vi "Create Oneof Message Converter Skeletons.vi"(8 "error in (no error)":errorcluster, 10 "Message parameters":T1[](array[typedef]), 11 "Library in":refnum<vi>) -> (0 "error out":errorcluster, 3 "Library out":refnum<vi>)   [LabVIEW 2019, in "gRPC Template Creation Utility.lvlib"]
uses:
  gRPC Template Creation Utility.lvlib
  TypeDefs/Message Metadata (Scripting).ctl
  TypeDefs/Message Element Metadata (Scripting).ctl
  TypeDefs/Message Element Type.ctl
  OneOf Constants/OneOfConstantsEnum.ctl
  <vilib>/Utility/traverseref.llb/TRef TravTarget.ctl
  <vilib>/Utility/traverseref.llb/VI Scripting - Traverse.lvlib
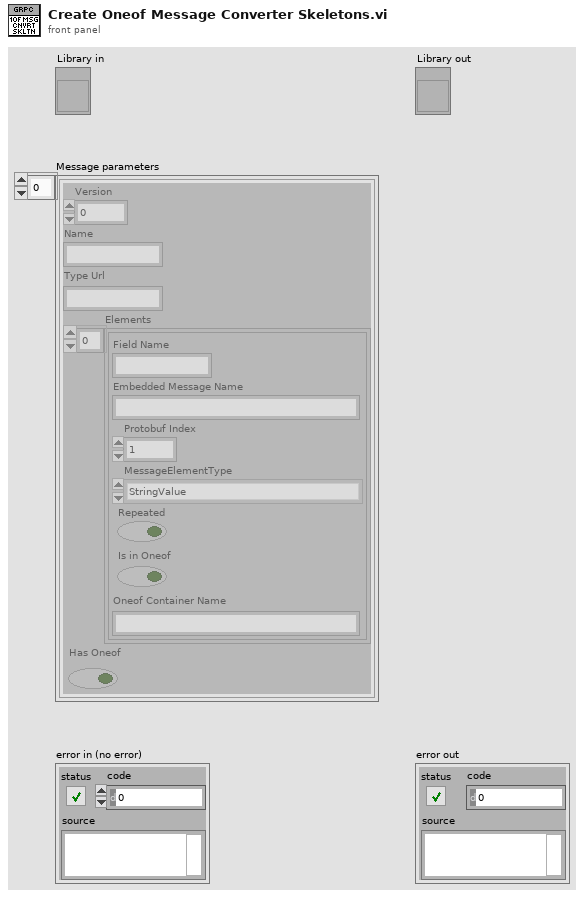
[diagram p1: front panel]
types:
  T1 = typedef "gRPC Template Creation Utility.lvlib/Message Metadata (Scripting).ctl" = cluster{"Version":i32, "Name":string, "Type Url":string, "Elements":T2[], "Has Oneof":bool}
  T2 = typedef "gRPC Template Creation Utility.lvlib/Message Element Metadata (Scripting).ctl" = cluster{"Field Name":string, "Embedded Message Name":string, "Protobuf Index":i32, "MessageElementType":T3, "Repeated":bool, "Is in Oneof":bool, "Oneof Container Name":string}
  T3 = typedef "gRPC Template Creation Utility.lvlib/Message Element Type.ctl" = enum32{"Int32Value", "FloatValue", "DoubleValue", "BoolValue", "StringValue", "MessageValue", "Int64Value", "UInt32Value", "UInt64Value", "EnumValue", "Bytes", "Fixed64", "Fixed32", "SFixed64", "SFixed32", "SInt64", "SInt32"}
  T4 = typedef "gRPC Template Creation Utility.lvlib/OneOfConstantsEnum.ctl" = enum16{"FlatToRichVIPrefix", "RichToFlatVIPrefix", "FlatTypeDefSuffix"}
  T5 = typedef "TRef TravTarget.ctl" = enum16{"FP", "BD", "Other"}
  T6 = enum32{"invalid scope", "public", "private", "protected", "community"}
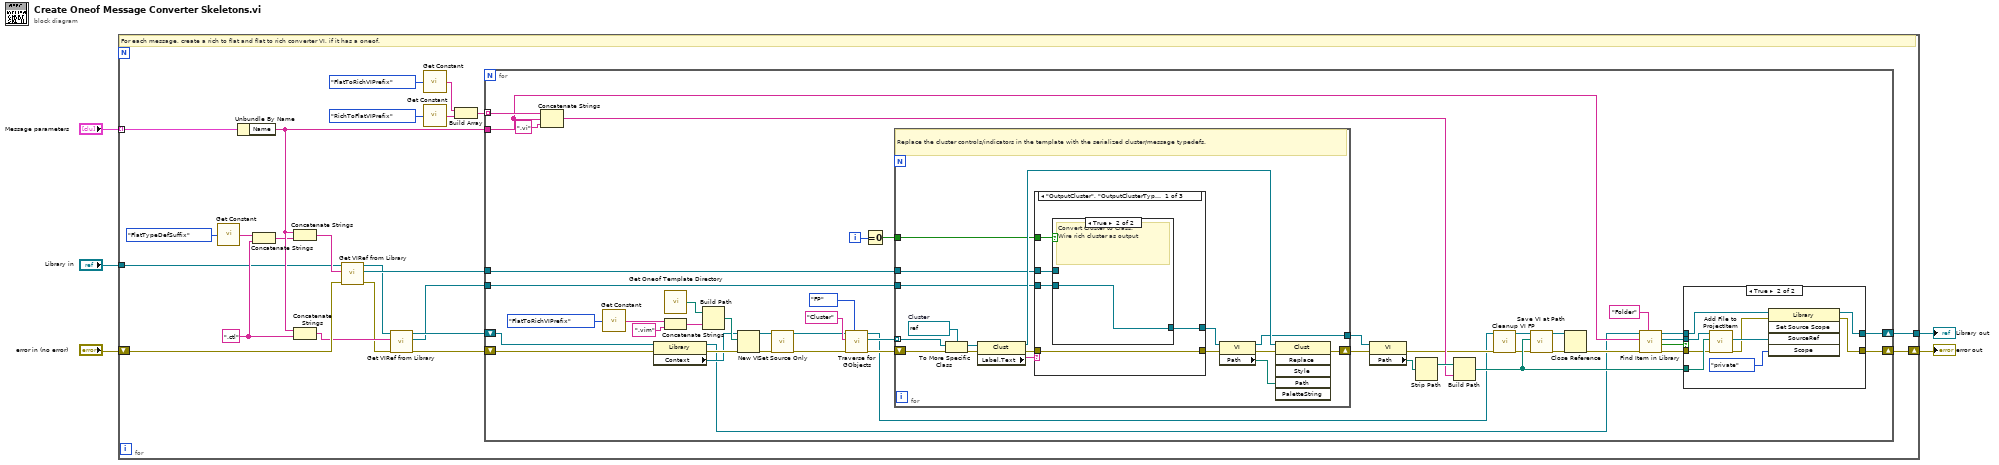
[diagram p0: block diagram]
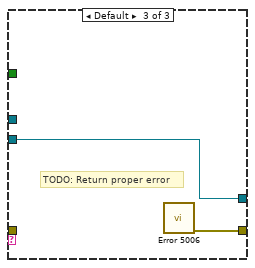
[diagram p6: hidden frame]
diagram:
  n1 = for {
    tunnel: "Message parameters" -> [w28] mode=indexing
    shift-right: [w23] -> w3
    shift-left: "error in (no error)" -> [w27]
    tunnel: "Library in" -> [w11]
    tunnel: [w25] -> w5
    w12 = ".ctl" ("string")
    # "For each message, create a rich to flat and flat to rich converter VI, if it has a oneof."
    n2 = call "Get Constant.vi"("Selection"=OneOfConstantsEnum."FlatTypeDefSuffix") -> ("String"=w18:string)
    n3 = Unbundle By Name(w28) -> ("Name"=w21:string)
    n4 = Concatenate Strings(w18, w12) -> (w20:string)
    n5 = Concatenate Strings(w21, w20) -> (w24:string)
    n6 = Concatenate Strings(w21, w12) -> (w22:string)
    n7 = call "Get VIRef from Library.vi"("error in (no error)"=w27, "Item Name"=w24, "Library"=w11) -> ("error out"=w7:errorcluster, "VIref out"=w9:refnum<vi>, "Library"=w8:refnum<vi>)  [unwired: 5 in, 1 out]
    n8 = call "Get VIRef from Library.vi"("error in (no error)"=w7, "Item Name"=w22, "Library"=w8) -> ("error out"=w6:errorcluster, "VIref out"=w10:refnum<vi>, "Library"=w26:refnum<vi>)  [unwired: 5 in, 1 out]
    n9 = call "Get Constant.vi"("Selection"=OneOfConstantsEnum."FlatToRichVIPrefix") -> ("String"=w15:string)
    n10 = call "Get Constant.vi"("Selection"=OneOfConstantsEnum."RichToFlatVIPrefix") -> ("String"=w14:string)
    n11 = Build Array(w15, w14) -> (w13:string[])
    n12 = for {
      tunnel: w9 -> [w74]
      tunnel: w21 -> [w51]
      tunnel: w10 -> [w68]
      shift-right: [w34] -> w25
      shift-left: w26 -> [w33]
      shift-right: [w55] -> w23
      shift-left: w6 -> [w32]
      tunnel: w13 -> [w62] mode=indexing
      i -> [w61]
      n13 = Concatenate Strings(w62, w51, ".vi" ("string")) -> (w69:string)
      n14 = call "Get Constant.vi"("Selection"=OneOfConstantsEnum."FlatToRichVIPrefix") -> ("String"=w49:string)
      n15 = property class="Library"(reference=w33, error in=w32) -> (reference out=w29:refnum<vi>, error out=w31:errorcluster, "Context"=w30:refnum<vi>)
      n16 = call "Get Oneof Template Directory.vi"() -> ("appended path"=w52:path)
      n17 = Concatenate Strings(w49, ".vim" ("string")) -> (w47:string)
      n18 = Build Path(base path=w52, name or relative path=w47) -> (appended path=w53:path)
      n19 = New VI(8:w31, 10:w53, 11:w30) -> (0:w46:errorcluster, 3:w44:refnum<vi>)  [unwired: 4 in]
      n20 = call "Set Source Only.vi"("error in (no error)"=w46, "VI in"=w44) -> ("error out"=w45:errorcluster, "VI out"=w43:refnum<vi>)  [unwired: 8 in]
      n21 = call <vilib>:"Traverse for GObjects.vi"("Traverse Target"=TRef_TravTarget."FP", "error in (no error)"=w45, "Class Name"="Cluster", "VI Refnum"=w43) -> ("error out"=w63:errorcluster, "References"=w65:refnum<vi>[], "dup VI Refnum"=w40:refnum<vi>)  [unwired: 4 in, 1 out]
      n22 = Equal To 0?(x=w61) -> (x = 0?=w60:bool)
      n23 = for {
        tunnel: w65 -> [w93] mode=indexing
        tunnel: w74 -> [w97]
        tunnel: w68 -> [w96]
        shift-right: [w92] -> w64
        shift-left: w63 -> [w94]
        tunnel: [w91] -> w73
        tunnel: w60 -> [w86]
        w101 = refnum<vi> refnum  # Cluster
        # "Replace the cluster controls/indicators in the template with the serialized cluster/message typedefs."
        n24 = To More Specific Class(target class=w101, reference=w93, error in=w94) -> (specific class reference=w100:refnum<vi>, error out=w102:errorcluster)
        n25 = property class="Clust"(reference=w100, error in=w102) -> (reference out=w98:refnum<vi>, error out=w95:errorcluster, "Label.Text"=w99:string)
        n26 = case shown="\"OutputCluster\", \"OutputClusterType\"" w99 {
          tunnel: w97 -> [w105 w113 _]
          tunnel: w96 -> [w104 w112 w117]
          tunnel: w95 -> [w107 w110 _]
          tunnel: [w103 w111 w117] -> w87
          tunnel: [w107 w110 w118] -> w88
          tunnel: w86 -> [w106 w114 _]
          frame "OutputCluster", "OutputClusterType" {
            n27 = case shown="True" w106 {
              tunnel: w105 -> [w108 _]
              tunnel: w104 -> [_ w109]
              tunnel: [w108 w109] -> w103
              frame False {
                # "Convert Class to Cluster. Wire flat cluster as output"
              }
              frame True {
                # "Convert Cluster to Class.\nWire rich cluster as output"
              }
            }
          }
          frame "InputCluster" {
            n28 = case shown="True" w114 {
              tunnel: w113 -> [_ w116]
              tunnel: w112 -> [w115 _]
              tunnel: [w115 w116] -> w111
              frame False {
                # "Convert Class to Cluster. Wire rich cluster as input."
              }
              frame True {
                # "Convert Cluster to Class. Wire flat cluster as input"
              }
            }
          }
          frame Default {
            # "TODO: Return proper error"
            n29 = call "Error 5006.vi"() -> ("error out"=w118:errorcluster)  [unwired: 11 in]
          }
        }
        n30 = property class="VI"(reference=w87, error in=w88) -> (reference out=w91:refnum<vi>, error out=w90:errorcluster, "Path"=w89:path)
        n31 = invoke class="Clust" method="Replace"(reference=w98, error in=w90, "Path"=w89) -> (error out=w92:errorcluster)  [unwired: 3 in, 5 out]
      }
      n32 = property class="VI"(reference=w73, error in=w64) -> (error out=w42:errorcluster, "Path"=w72:path)  [unwired: 1 out]
      n33 = Strip Path(path=w72) -> (stripped path=w71:path)  [unwired: 1 out]
      n34 = Build Path(base path=w71, name or relative path=w69) -> (appended path=w57:path)
      n35 = call "Cleanup VI FP.vi"("error in"=w42, "vi in"=w40) -> ("error out"=w41:errorcluster, "vi out"=w39:refnum<vi>)  [unwired: 8 in]
      n36 = call "Save VI at Path.vi"("error in (no error)"=w41, "Path"=w57, "VI in"=w39) -> ("error out"=w38:errorcluster, "VI out"=w37:refnum<vi>)  [unwired: 6 in, 1 out]
      n37 = Close Reference(reference=w37, error in (no error)=w38) -> (error out=w36:errorcluster)
      n38 = call "Find Item in Library.vi"("Item Type"="Folder", "error in (no error)"=w36, "Item Name"=w51, "Library item in"=w29) -> ("error out"=w56:errorcluster, "Found?"=w54:bool, "Project Item (Library Item)"=w58:refnum<vi>, "Library item out"=w35:refnum<vi>)  [unwired: 4 in]
      n39 = case shown="True" w54 {
        tunnel: w58 -> [_ w85]
        tunnel: w57 -> [_ w84]
        tunnel: w56 -> [w76 w83]
        tunnel: [w76 w78] -> w55
        tunnel: w35 -> [w75 w82]
        tunnel: [w75 w80] -> w34
        frame False {
        }
        frame True {
          n40 = call "Add File to ProjectItem.vi"("error in (no error)"=w83, "File Path"=w84, "ProjectItem in"=w85) -> ("error out"=w79:errorcluster, "Added File ref"=w81:refnum<vi>)  [unwired: 6 in, 1 out]
          n41 = invoke class="Library" method="Set Source Scope"(reference=w82, error in=w79, "SourceRef"=w81, "Scope"=T6."private" ("scope")) -> (reference out=w80:refnum<vi>, error out=w78:errorcluster)  [unwired: 1 in, 3 out]
        }
      }
    }
  }
  "Library out" <- w5
  "error out" <- w3
